vi "Close.vi"(8 "error in (no error)":errorcluster, 11 "Session in":refnum<class "Session.lvclass">) -> (0 "error out":errorcluster)   [LabVIEW 2020]
doc: "Performs an instrument error query before terminating the software connection to the instrument."
uses:
  CTI/Session/Session.lvclass
panel:
  # "Input"
  # "Output"
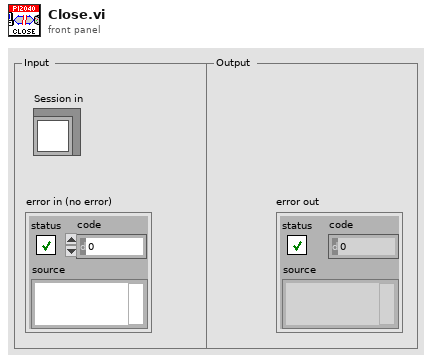
[diagram p1: front panel]
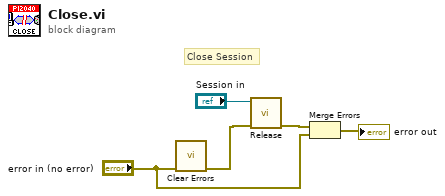
[diagram p0: block diagram]
diagram:
  # "Close Session"
  n1 = call <vilib>:"Clear Errors.vi"("error in (no error)"="error in (no error)") -> ("error out"=w3:errorcluster)  [unwired: 5 in, 1 out]
  n2 = call-dynamic "Release.vi"("error in (no error)"=w3, "Session in"="Session in") -> ("error out"=w2:errorcluster)  [unwired: 9 in]
  n3 = Merge Errors(w2, "error in (no error)") -> (→"error out":errorcluster)
